vi "Load XML.vi"(8 "error in":errorcluster, 10 "XML":string, 11 "XML Document in":refnum<k24>) -> (0 "error out":errorcluster, 3 "XML Document out":refnum<k24>)   [LabVIEW 2026, in "ToastNotification.lvlib" / "Toast Native.lvlib"]
doc: "Load XML into a borrowed WinRT XML Document using its LoadXml method. Skipped on incoming error. XML Document out aliases the input; the caller remains its owner. Release the boxed string, invocation result and reflection metadata even on failure. A parse failure does not promise rollback of the document. Parsing is not full toast-schema validation."
uses:
  Toast Native.lvlib
  Reflection DotNet/Reflection DotNet.lvlib
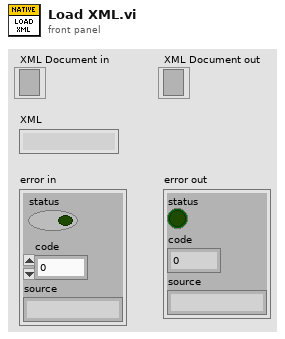
[diagram p1: front panel]
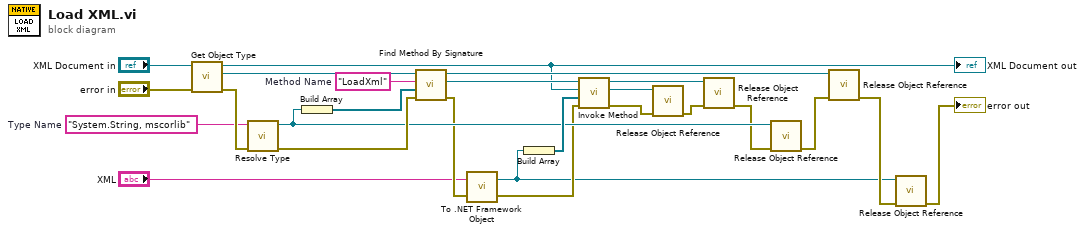
[diagram p0: block diagram]
diagram:
  w18 = "LoadXml"  # Method Name
  w22 = "System.String, mscorlib"  # Type Name
  n1 = call "Get Object Type.vi"("error in (no error)"="error in", "Object in"="XML Document in") -> ("error out"=w23:errorcluster, "Object Type"=w21:refnum<k24>, "Object out"=w9:refnum<k24>)  [unwired: 7 in]
  "XML Document out" <- w9
  n2 = call "Resolve Type.vi"("error in"=w23, "Type Name"=w22) -> ("error out"=w20:errorcluster, "Runtime Type"=w14:refnum<k24>)  [unwired: 8 in]
  n3 = Build Array(w14) -> (w19:refnum<k24>[])
  n4 = call "Find Method By Signature.vi"("error in"=w20, "Parameter Types"=w19, "Method Name"=w18, "Declaring Type in"=w21) -> ("error out"=w4:errorcluster, "Method Info"=w17:refnum<k24>, "Declaring Type out"=w12:refnum<k24>)  [unwired: 5 in]
  n5 = call <vilib>:"To .NET Framework Object.vi"("error in (no error)"=w4, "anything"="XML") -> ("error out"=w3:errorcluster, ".NET object"=w2:refnum<k24>)
  n6 = Build Array(w2) -> (w16:refnum<k24>[])
  n7 = call "Invoke Method.vi"("error in (no error)"=w3, "parameters"=w16, "Target Object"=w9, "Method Info in"=w17) -> ("error out"=w8:errorcluster, "Return Value"=w7:refnum<k24>, "Method Info out"=w15:refnum<k24>)  [unwired: 5 in]
  n8 = call "Release Object Reference.vi"("error in"=w8, "object"=w7) -> ("error out"=w6:errorcluster)  [unwired: 9 in]
  n9 = call "Release Object Reference.vi"("error in"=w6, "object"=w15) -> ("error out"=w13:errorcluster)  [unwired: 9 in]
  n10 = call "Release Object Reference.vi"("error in"=w13, "object"=w14) -> ("error out"=w11:errorcluster)  [unwired: 9 in]
  n11 = call "Release Object Reference.vi"("error in"=w11, "object"=w12) -> ("error out"=w10:errorcluster)  [unwired: 9 in]
  n12 = call "Release Object Reference.vi"("error in"=w10, "object"=w2) -> ("error out"=→"error out":errorcluster)  [unwired: 9 in]
